vi "Process Messages.vi"(8 "error in (no error)":errorcluster, 11 "Deck in":refnum<class "Deck.lvclass">) -> (0 "error out":errorcluster, 3 "Deck out":refnum<class "Deck.lvclass">)   [LabVIEW 2019, in "Deck.lvclass"]
uses:
  Deck.lvclass
  Deck.lvclass/Deck.ctl
  Libraries/Track Info/Track Info.ctl
  State.ctl
  Packed Libraries/Messaging.lvlibp/Message Cluster.ctl
  Libraries/Track Info/Track Info FGV Enum.ctl
  Packed Libraries/Globals.lvlibp/Constants.vi
  Libraries/Audio File Input/Audio File Input.lvlib
  Packed Libraries/Messaging.lvlibp
  Libraries/User Interface/User Interface.lvlib
  Libraries/Track Info/Track Info.lvlib
  Packed Libraries/Globals.lvlibp
  Packed Libraries/Audio Processing.lvlibp
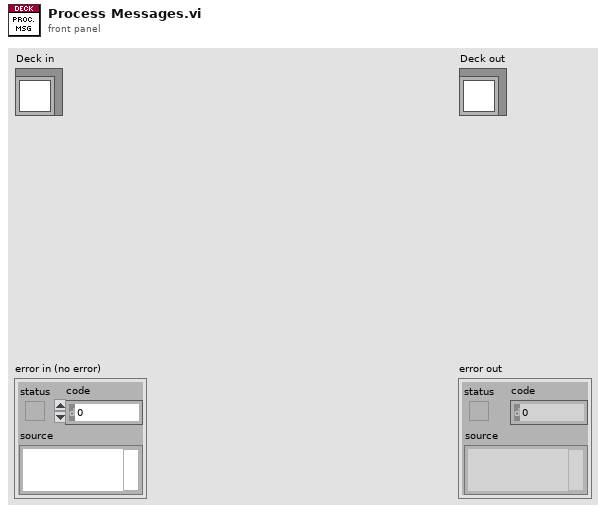
[diagram p1: front panel]
types:
  T1 = typedef "Track Info.lvlib/Track Info.ctl" = cluster{"Path":path, "Length (Samples)":i32, "Channels":i32, "Sample Rate (Hz)":i32, "BPM":dbl, "Cue Points (Samples)":i32[]}
  T2 = typedef "Messaging.lvlibp/Message Cluster.ctl" = cluster{"Event":string, "Source":string, "Target":string, "Data":variant}
  T3 = typedef "Deck.lvclass/State.ctl" = enum16{"No Track", "Loading", "Active", "Scratching", "Brake", "Backspin"}
  T4 = typedef "Track Info.lvlib/Track Info FGV Enum.ctl" = enum16{"Init", "Update Track", "Update Multiple Tracks", "Get Track", "Get Multiple Tracks"}
  T5 = typedef "Audio Processing.lvlibp/Value Properties.ctl" = cluster{"Lower":dbl, "Upper":dbl, "Default":dbl, "Increment":dbl}
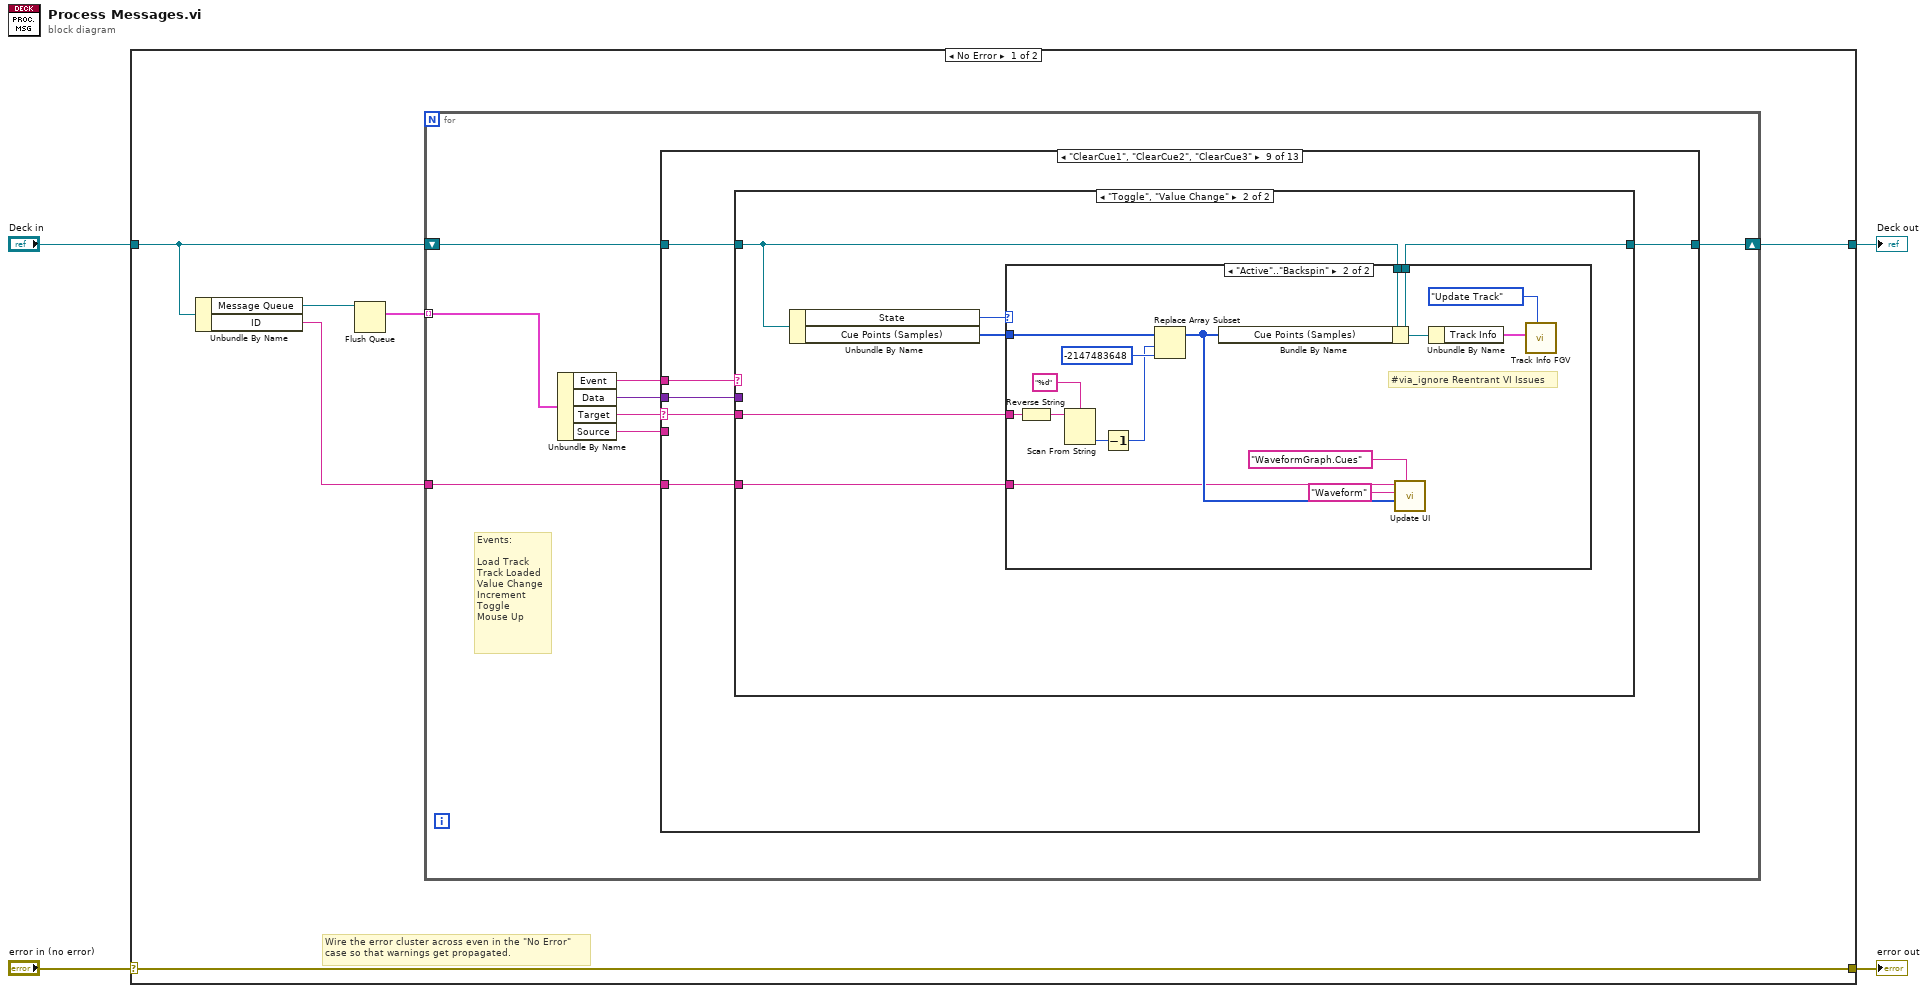
[diagram p0: block diagram]
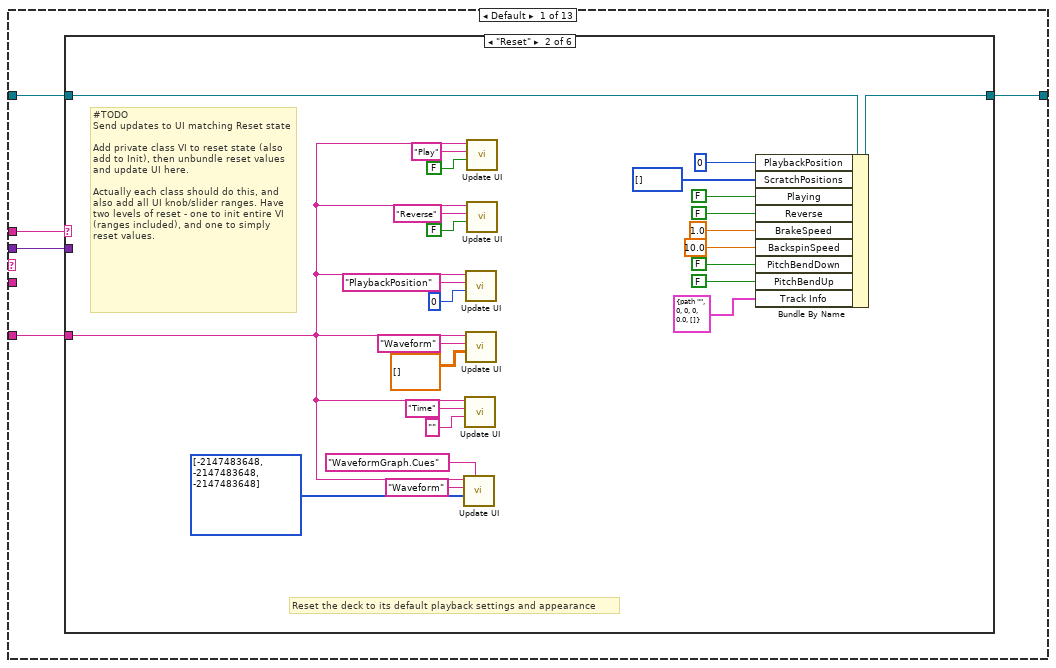
[diagram p2: hidden frame]
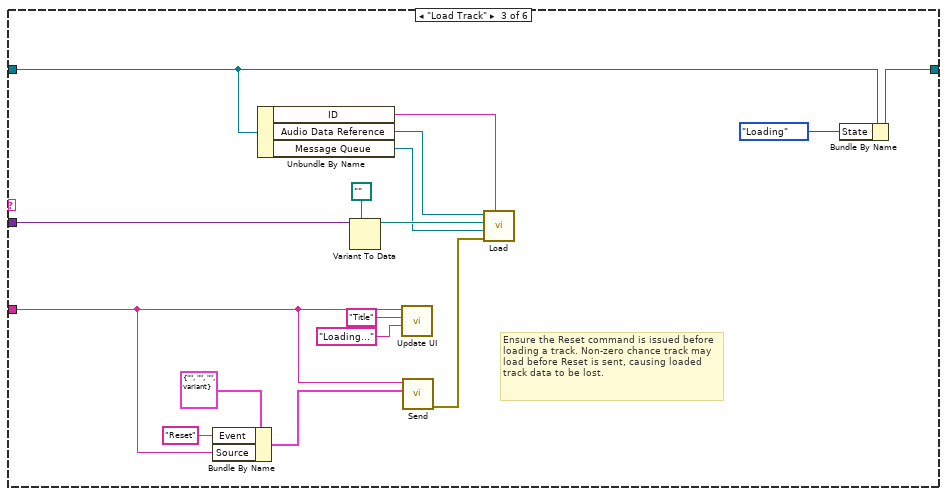
[diagram p4: hidden frame]
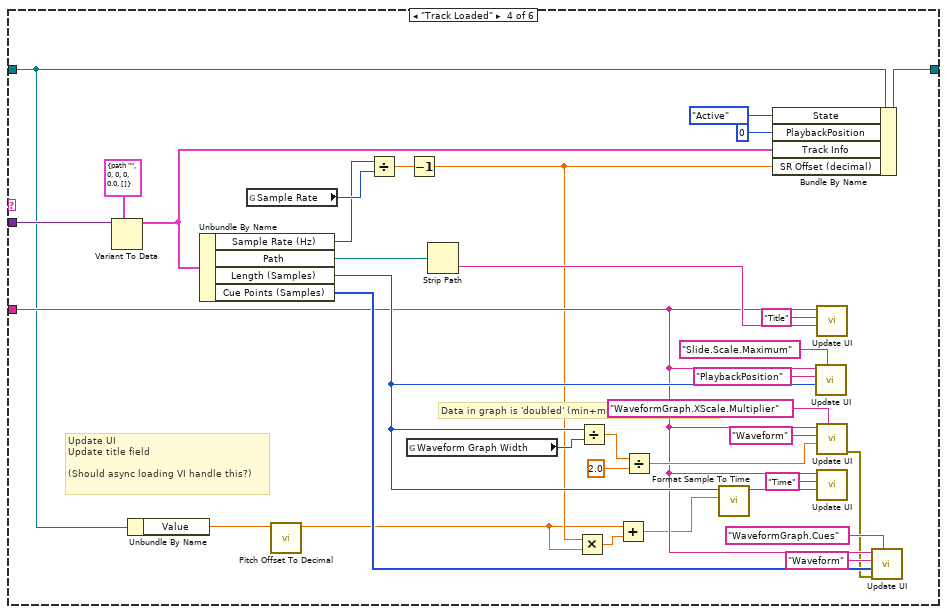
[diagram p5: hidden frame]
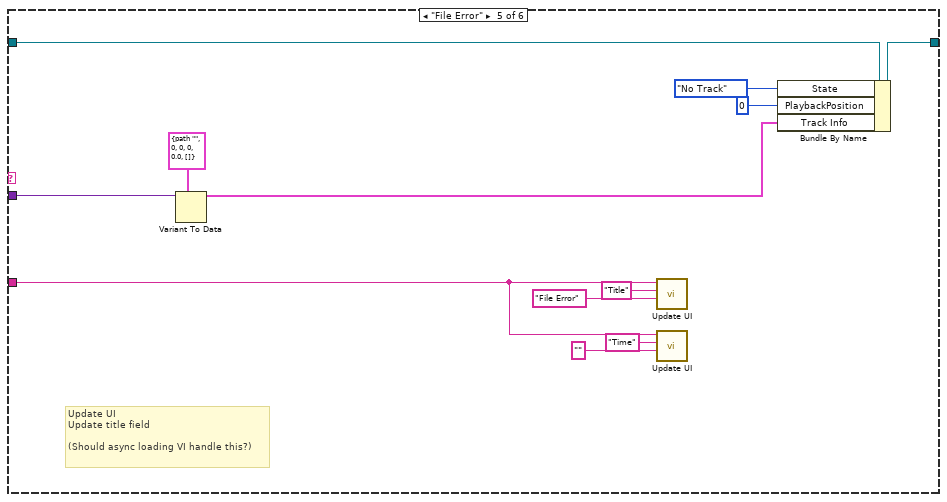
[diagram p6: hidden frame]
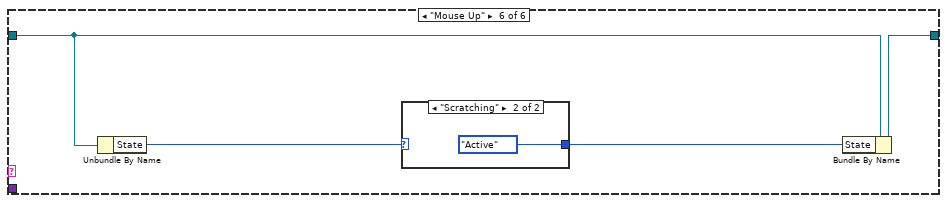
[diagram p7: hidden frame]
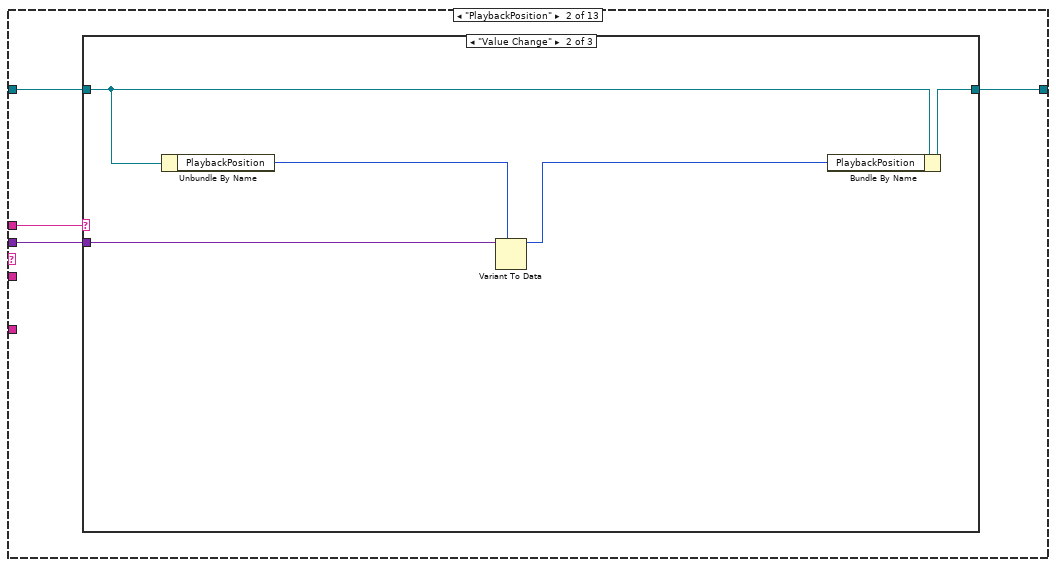
[diagram p9: hidden frame]
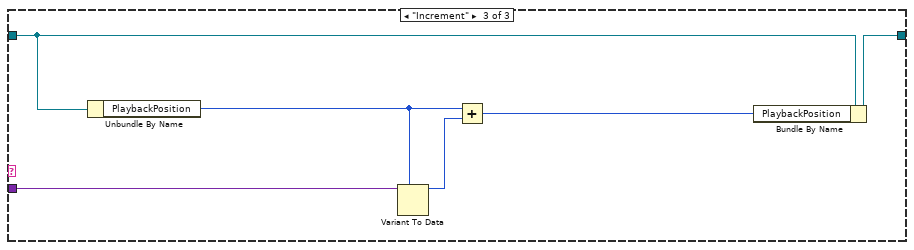
[diagram p11: hidden frame]
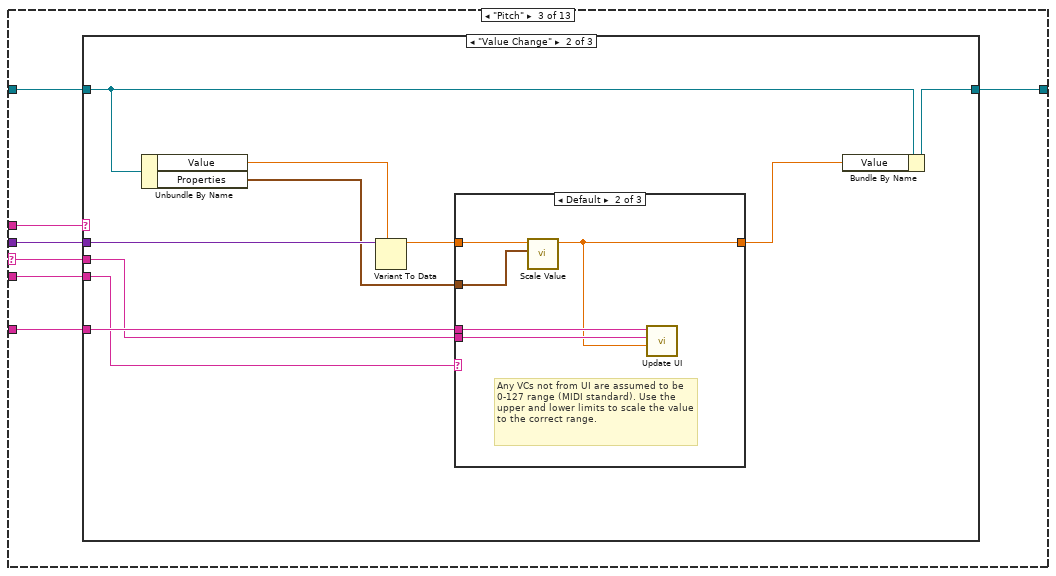
[diagram p12: hidden frame]
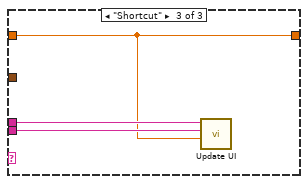
[diagram p15: hidden frame]
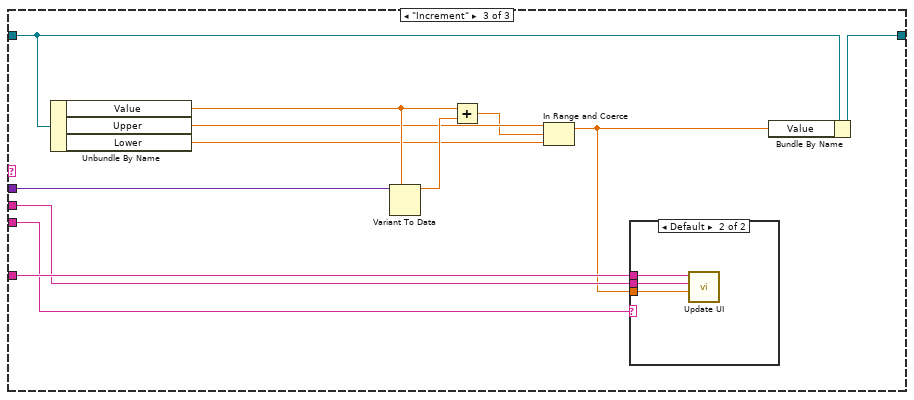
[diagram p16: hidden frame]
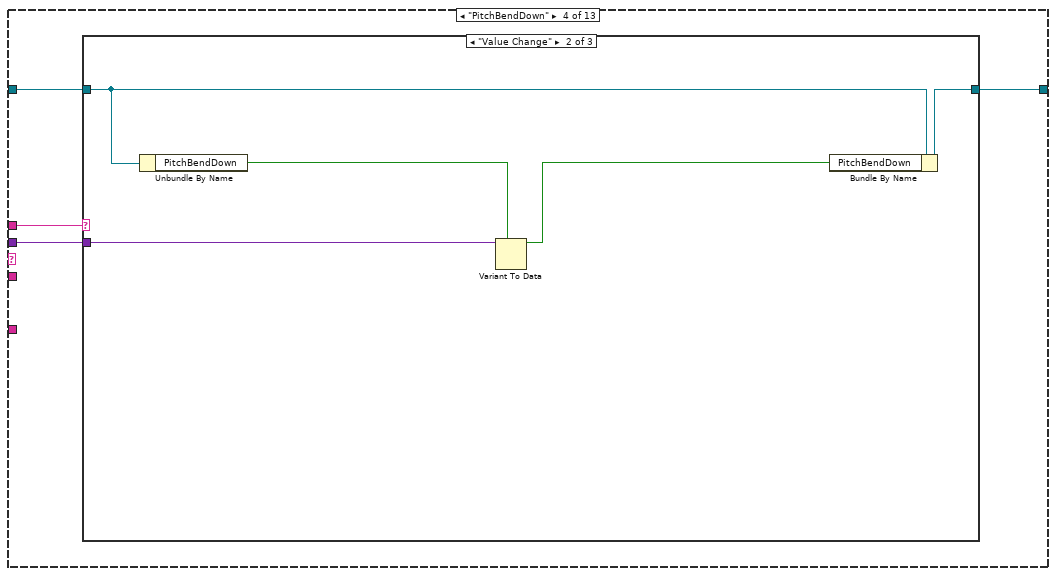
[diagram p18: hidden frame]
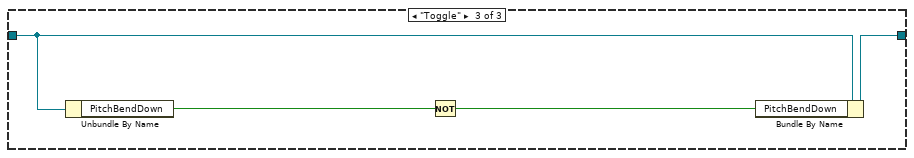
[diagram p20: hidden frame]
diagram:
  n1 = case shown="No Error" "error in (no error)" {
    selector: "error in (no error)" -> [w10 w558]
    tunnel: [w10 w558] -> w3
    tunnel: [w9 w557] -> w1
    tunnel: "Deck in" -> [w8 w557]
    frame No Error {
      # "Wire the error cluster across even in the \"No Error\"\ncase so that warnings get propagated."
      n2 = Unbundle By Name(w8) -> ("Message Queue"=w6:refnum<queue>, "ID"=w7:string)
      n3 = Flush Queue(queue=w6) -> (remaining elements=w5:T2[])  [unwired: 1 in, 2 out]
      n4 = for {
        shift-right: [w16] -> w9
        shift-left: w8 -> [w18]
        tunnel: w7 -> [w14]
        tunnel: w5 -> [w11] mode=indexing
        # "Events:\n\nLoad Track\nTrack Loaded\nValue Change\nIncrement\nToggle\nMouse Up"
        n5 = Unbundle By Name(w11) -> ("Event"=w17:string, "Data"=w15:variant, "Target"=w13:string, "Source"=w12:string)
        n6 = case shown="\"ClearCue1\", \"ClearCue2\", \"ClearCue3\"" w13 {
          selector: w13 -> [_ _ w135 _ _ _ w223 w250 w280 w310 w347 w377 w468]
          tunnel: w18 -> [w23 w121 w140 w179 w193 w207 w227 w254 w284 w314 w352 w381 w472]
          tunnel: w17 -> [w22 w120 w139 w178 w192 w206 w226 w253 w283 w313 w351 w380 w471]
          tunnel: [w21 w119 w138 w177 w191 w205 w225 w252 w282 w312 w350 w379 w470] -> w16
          tunnel: w15 -> [w20 w118 w137 w176 w190 w204 w224 w251 w281 w311 w349 w378 w469]
          tunnel: w14 -> [w19 _ w136 _ _ _ _ w249 w279 w309 w348 w376 w467]
          tunnel: w12 -> [_ _ w134 _ _ _ _ _ _ w308 w346 w375 w466]
          frame Default {
            n7 = case shown="\"Reset\"" w22 {
              tunnel: w23 -> [w24 w42 w58 w71 w109 w112]
              tunnel: [w24 w43 w59 w97 w108 w113] -> w21
              tunnel: w20 -> [_ _ w57 w96 w107 _]
              tunnel: w19 -> [_ w27 w51 w76 w103 _]
              frame Default {
              }
              frame "Reset" {
                # "#TODO\nSend updates to UI matching Reset state\n\nAdd private class VI to reset state (also add to Init), then unbundle reset values and update UI here.\n\nActually each class should do this, and also add all UI knob/slider ranges. Have two levels of reset - one to init entire VI (ranges included), and one to simply reset values."
                # "Reset the deck to its default playback settings and appearance"
                n8 = call "Update UI.vi"("Message (Value Change)"="WaveformGraph.Cues" ("format string"), "Data"=i32[] [-2147483648, -2147483648, -2147483648] ("Cue Points (Samples)"), "Target"="Waveform", "ID"=w27) -> ()  [unwired: 7 in, 1 out]
                n9 = call "Update UI.vi"("Data"="" ("Target"), "Target"="Time", "ID"=w27) -> ()  [unwired: 8 in, 1 out]
                n10 = call "Update UI.vi"("Data"=0, "Target"="PlaybackPosition", "ID"=w27) -> ()  [unwired: 8 in, 1 out]
                n11 = call "Update UI.vi"("Data"=dbl[][] [], "Target"="Waveform", "ID"=w27) -> ()  [unwired: 8 in, 1 out]
                n12 = call "Update UI.vi"("Data"=FALSE ("Playing"), "Target"="Play", "ID"=w27) -> ()  [unwired: 8 in, 1 out]
                n13 = call "Update UI.vi"("Data"=FALSE ("Playing"), "Target"="Reverse", "ID"=w27) -> ()  [unwired: 8 in, 1 out]
                n14 = Bundle By Name(cluster=w42, "PlaybackPosition"=0, "ScratchPositions"=i32[] [], "Playing"=FALSE, "Reverse"=FALSE, "BrakeSpeed"=1.0, "BackspinSpeed"=10.0, "PitchBendDown"=FALSE, "PitchBendUp"=FALSE, "Track Info"=T1 {"Path"=path "", "Length (Samples)"=0, "Channels"=0, "Sample Rate (Hz)"=0, "BPM"=0.0, "Cue Points (Samples)"=[]}) -> (w43:refnum<class "Deck.lvclass">)
              }
              frame "Load Track" {
                # "Ensure the Reset command is issued before loading a track. Non-zero chance track may load before Reset is sent, causing loaded track data to be lost."
                n15 = Bundle By Name(cluster=T2 {"Event"="", "Source"="", "Target"="", "Data"=variant} ("Message"), "Event"="Reset", "Source"=w51) -> (w52:T2)
                n16 = Unbundle By Name(w58) -> ("ID"=w65:string, "Audio Data Reference"=w62:refnum<data-value>, "Message Queue"=w61:refnum<queue>)
                n17 = Variant To Data(type=path "", Variant=w57) -> (data=w64:path)  [unwired: 1 in, 1 out]
                n18 = call "Update UI.vi"("Data"="Loading..." ("Target"), "Target"="Title", "ID"=w51) -> ()  [unwired: 8 in, 1 out]
                n19 = call "Send.vi"("Message"=w52, "Queue Name"=w51) -> ("error out"=w50:errorcluster)  [unwired: 9 in]
                n20 = call "Load.vi"("Deck ID"=w65, "error in (no error)"=w50, "Message Queue"=w61, "Path"=w64, "Audio Data Reference"=w62) -> ()  [unwired: 6 in, 1 out]
                n21 = Bundle By Name(cluster=w58, "State"=State."Loading") -> (w59:refnum<class "Deck.lvclass">)
              }
              frame "Track Loaded" {
                # "Data in graph is 'doubled' (min+max for every point)"
                # "Update UI\nUpdate title field\n\n(Should async loading VI handle this?)"
                n22 = Variant To Data(type=T1 {"Path"=path "", "Length (Samples)"=0, "Channels"=0, "Sample Rate (Hz)"=0, "BPM"=0.0, "Cue Points (Samples)"=[]} ("Track Info"), Variant=w96) -> (data=w94:T1)  [unwired: 1 in, 1 out]
                n23 = Unbundle By Name(w71) -> ("Value"=w70:dbl)
                n24 = Unbundle By Name(w94) -> ("Sample Rate (Hz)"=w72:i32, "Path"=w93:path, "Length (Samples)"=w84:i32, "Cue Points (Samples)"=w77:i32[])
                n25 = global read "Constants.vi" "Sample Rate"() -> (w74:i32)
                n26 = call "Pitch Offset To Decimal.vi"("Pitch Offset (%)"=w70) -> ("Pitch (decimal)"=w67:dbl)  [unwired: 10 in]
                n27 = Divide(x=w72, y=w74) -> (x/y=w73:dbl)
                n28 = global read "Constants.vi" "Waveform Graph Width"() -> (w83:i32)
                n29 = Decrement(x=w73) -> (x-1=w68:dbl)
                n30 = Strip Path(path=w93) -> (name=w92:string)  [unwired: 1 out]
                n31 = Multiply(x=w68, y=w67) -> (x*y=w69:dbl)
                n32 = Divide(x=w84, y=w83) -> (x/y=w82:dbl)
                n33 = Add(x=w67, y=w69) -> (x+y=w66:dbl)
                n34 = Divide(x=w82, y=2.0 ("x")) -> (x/y=w80:dbl)
                n35 = call "Format Sample To Time.vi"("Pitch (decimal) (1)"=w66, "Samples"=w84) -> ("Formatted Time"=w88:string)  [unwired: 9 in]
                n36 = Bundle By Name(cluster=w71, "State"=State."Active", "PlaybackPosition"=0 ("Playback Position (Samples)"), "Track Info"=w94, "SR Offset (decimal)"=w68) -> (w97:refnum<class "Deck.lvclass">)
                n37 = call "Update UI.vi"("Message (Value Change)"="Slide.Scale.Maximum" ("Target"), "Data"=w84, "Target"="PlaybackPosition", "ID"=w76) -> ()  [unwired: 7 in, 1 out]
                n38 = call "Update UI.vi"("Data"=w92, "Target"="Title", "ID"=w76) -> ()  [unwired: 8 in, 1 out]
                n39 = call "Update UI.vi"("Message (Value Change)"="WaveformGraph.XScale.Multiplier" ("Target"), "Data"=w80, "Target"="Waveform", "ID"=w76) -> ("error out"=w75:errorcluster)  [unwired: 7 in]
                n40 = call "Update UI.vi"("Data"=w88, "Target"="Time", "ID"=w76) -> ()  [unwired: 8 in, 1 out]
                n41 = call "Update UI.vi"("Message (Value Change)"="WaveformGraph.Cues" ("format string"), "error in (no error)"=w75, "Data"=w77, "Target"="Waveform", "ID"=w76) -> ()  [unwired: 6 in, 1 out]
              }
              frame "File Error" {
                # "Update UI\nUpdate title field\n\n(Should async loading VI handle this?)"
                n42 = Variant To Data(type=T1 {"Path"=path "", "Length (Samples)"=0, "Channels"=0, "Sample Rate (Hz)"=0, "BPM"=0.0, "Cue Points (Samples)"=[]} ("Track Info"), Variant=w107) -> (data=w105:T1)  [unwired: 1 in, 1 out]
                n43 = call "Update UI.vi"("Data"="File Error" ("Target"), "Target"="Title", "ID"=w103) -> ()  [unwired: 8 in, 1 out]
                n44 = call "Update UI.vi"("Data"="" ("Target"), "Target"="Time", "ID"=w103) -> ()  [unwired: 8 in, 1 out]
                n45 = Bundle By Name(cluster=w109, "State"=State."No Track", "PlaybackPosition"=0 ("Playback Position (Samples)"), "Track Info"=w105) -> (w108:refnum<class "Deck.lvclass">)
              }
              frame "Mouse Up" {
                n46 = Unbundle By Name(w112) -> ("State"=w114:T3)
                n47 = case shown="\"Scratching\"" w114 {
                  selector: w114 -> [w116 _]
                  tunnel: [w116 State."Active" ("State")] -> w115
                  frame Default {
                  }
                  frame "Scratching" {
                  }
                }
                n48 = Bundle By Name(cluster=w112, "State"=w115) -> (w113:refnum<class "Deck.lvclass">)
              }
            }
          }
          frame "PlaybackPosition" {
            n49 = case shown="\"Value Change\"" w120 {
              tunnel: w121 -> [w122 w126 w132]
              tunnel: [w122 w127 w133] -> w119
              tunnel: w118 -> [_ w124 w131]
              frame Default {
              }
              frame "Value Change" {
                n50 = Unbundle By Name(w126) -> ("PlaybackPosition"=w125:i32)
                n51 = Variant To Data(type=w125, Variant=w124) -> (data=w123:i32)  [unwired: 1 in, 1 out]
                n52 = Bundle By Name(cluster=w126, "PlaybackPosition"=w123) -> (w127:refnum<class "Deck.lvclass">)
              }
              frame "Increment" {
                n53 = Unbundle By Name(w132) -> ("PlaybackPosition"=w130:i32)
                n54 = Variant To Data(type=w130, Variant=w131) -> (data=w129:i32)  [unwired: 1 in, 1 out]
                n55 = Add(x=w130, y=w129) -> (x+y=w128:i32)
                n56 = Bundle By Name(cluster=w132, "PlaybackPosition"=w128) -> (w133:refnum<class "Deck.lvclass">)
              }
            }
          }
          frame "Pitch" {
            n57 = case shown="\"Value Change\"" w139 {
              tunnel: w140 -> [w141 w150 w171]
              tunnel: [w141 w151 w172] -> w138
              tunnel: w137 -> [_ w148 w170]
              tunnel: w136 -> [_ w147 w167]
              tunnel: w135 -> [_ w145 w166]
              tunnel: w134 -> [_ w144 w165]
              frame Default {
              }
              frame "Value Change" {
                n58 = Unbundle By Name(w150) -> ("Value"=w149:dbl, "Properties"=w142:T5)
                n59 = Variant To Data(type=w149, Variant=w148) -> (data=w146:dbl)  [unwired: 1 in, 1 out]
                n60 = case shown="Default" w144 {
                  tunnel: w147 -> [_ w157 w160]
                  tunnel: w145 -> [_ w156 w159]
                  tunnel: w146 -> [w152 w153 w158]
                  tunnel: [w152 w154 w158] -> w143
                  tunnel: w142 -> [_ w155 _]
                  frame "UI" {
                    # "VC from UI are assumed to be in range."
                  }
                  frame Default {
                    # "Any VCs not from UI are assumed to be 0-127 range (MIDI standard). Use the upper and lower limits to scale the value to the correct range."
                    n61 = call "Scale Value.vi"("Properties"=w155, "Value"=w153) -> ("Scaled Value"=w154:dbl)  [unwired: 9 in]
                    n62 = call "Update UI.vi"("Data"=w154, "Target"=w156, "ID"=w157) -> ()  [unwired: 8 in, 1 out]
                  }
                  frame "Shortcut" {
                    n63 = call "Update UI.vi"("Data"=w158, "Target"=w159, "ID"=w160) -> ()  [unwired: 8 in, 1 out]
                  }
                }
                n64 = Bundle By Name(cluster=w150, "Value"=w143) -> (w151:refnum<class "Deck.lvclass">)
              }
              frame "Increment" {
                n65 = Unbundle By Name(w171) -> ("Value"=w169:dbl, "Upper"=w164:dbl, "Lower"=w163:dbl)
                n66 = Variant To Data(type=w169, Variant=w170) -> (data=w168:dbl)  [unwired: 1 in, 1 out]
                n67 = Add(x=w169, y=w168) -> (x+y=w162:dbl)
                n68 = In Range and Coerce(upper limit=w164, x=w162, lower limit=w163) -> (coerced(x)=w161:dbl)  [unwired: 1 out]
                n69 = case shown="Default" w165 {
                  tunnel: w167 -> [_ w175]
                  tunnel: w166 -> [_ w174]
                  tunnel: w161 -> [_ w173]
                  frame "UI" {
                  }
                  frame Default {
                    n70 = call "Update UI.vi"("Data"=w173, "Target"=w174, "ID"=w175) -> ()  [unwired: 8 in, 1 out]
                  }
                }
                n71 = Bundle By Name(cluster=w171, "Value"=w161) -> (w172:refnum<class "Deck.lvclass">)
              }
            }
          }
          frame "PitchBendDown" {
            n72 = case shown="\"Value Change\"" w178 {
              tunnel: w179 -> [w180 w184 w188]
              tunnel: [w180 w185 w189] -> w177
              tunnel: w176 -> [_ w182 _]
              frame Default {
              }
              frame "Value Change" {
                n73 = Unbundle By Name(w184) -> ("PitchBendDown"=w183:bool)
                n74 = Variant To Data(type=w183, Variant=w182) -> (data=w181:bool)  [unwired: 1 in, 1 out]
                n75 = Bundle By Name(cluster=w184, "PitchBendDown"=w181) -> (w185:refnum<class "Deck.lvclass">)
              }
              frame "Toggle" {
                n76 = Unbundle By Name(w188) -> ("PitchBendDown"=w187:bool)
                n77 = Not(x=w187) -> (.not. x?=w186:bool)
                n78 = Bundle By Name(cluster=w188, "PitchBendDown"=w186) -> (w189:refnum<class "Deck.lvclass">)
              }
            }
          }
          frame "PitchBendUp" {
            n79 = case shown="\"Value Change\"" w192 {
              tunnel: w193 -> [w194 w198 w202]
              tunnel: [w194 w199 w203] -> w191
              tunnel: w190 -> [_ w196 _]
              frame Default {
              }
              frame "Value Change" {
                n80 = Unbundle By Name(w198) -> ("PitchBendUp"=w197:bool)
                n81 = Variant To Data(type=w197, Variant=w196) -> (data=w195:bool)  [unwired: 1 in, 1 out]
                n82 = Bundle By Name(cluster=w198, "PitchBendUp"=w195) -> (w199:refnum<class "Deck.lvclass">)
              }
              frame "Toggle" {
                n83 = Unbundle By Name(w202) -> ("PitchBendUp"=w201:bool)
                n84 = Not(x=w201) -> (.not. x?=w200:bool)
                n85 = Bundle By Name(cluster=w202, "PitchBendUp"=w200) -> (w203:refnum<class "Deck.lvclass">)
              }
            }
          }
          frame "Jogwheel" {
            n86 = case shown="\"Value Change\"" w206 {
              tunnel: w207 -> [w208 w219]
              tunnel: [w208 w220] -> w205
              tunnel: w204 -> [_ w218]
              frame Default {
              }
              frame "Value Change" {
                n87 = Unbundle By Name(w219) -> ("State"=w217:T3, "ScratchPositions"=w214:i32[], "PlaybackPosition"=w212:i32)
                n88 = Variant To Data(type=w212, Variant=w218) -> (data=w211:i32)  [unwired: 1 in, 1 out]
                n89 = Subtract(x=w214, y=w212) -> (x-y=w215:i32[])
                n90 = case shown="\"Active\"" w217 {
                  selector: w217 -> [w221 _]
                  tunnel: [w221 State."Scratching" ("State")] -> w216
                  frame Default {
                  }
                  frame "Active" {
                  }
                }
                n91 = Add Array Elements(numeric array=w215) -> (sum=w213:i32)
                n92 = Compound Arithmetic op=ADD(w213, w212, w211) -> (w210:i32)
                n93 = Build Array(w210) -> (w209:i32[])
                n94 = Bundle By Name(cluster=w219, "State"=w216, "ScratchPositions"=w209) -> (w220:refnum<class "Deck.lvclass">)
              }
            }
          }
          frame "Cue1", "Cue2", "Cue3" {
            n95 = case shown="\"Toggle\", \"Value Change\"" w226 {
              tunnel: w227 -> [w228 w232]
              tunnel: [w228 w233] -> w225
              tunnel: w224 -> [_ _]
              tunnel: w223 -> [_ w230]
              frame Default {
              }
              frame "Toggle", "Value Change" {
                n96 = Unbundle By Name(w232) -> ("State"=w229:T3, "Cue Points (Samples)"=w231:i32[])
                n97 = case shown="\"Active\"..\"Backspin\"" w229 {
                  tunnel: [w234 w244] -> w233
                  tunnel: w232 -> [w234 w243]
                  tunnel: w231 -> [_ w242]
                  tunnel: w230 -> [_ w237]
                  frame Default {
                  }
                  frame "Active".."Backspin" {
                    n98 = Reverse String(1:w237) -> (0:w239:string)
                    n99 = Scan From String(format string="%d", input string=w239) -> (output 1=w236:i32)  [unwired: 3 in, 3 out]
                    n100 = Decrement(x=w236) -> (x-1=w235:i32)
                    n101 = Index Array(array=w242, index=w235) -> (element=w240:i32)
                    n102 = Greater Or Equal To 0?(x=w240) -> (x >= 0?=w241:bool)
                    n103 = case shown="True" w241 {
                      tunnel: [w245 w248] -> w244
                      tunnel: w243 -> [w245 w247]
                      tunnel: w240 -> [_ w246]
                      frame False {
                      }
                      frame True {
                        n104 = Bundle By Name(cluster=w247, "PlaybackPosition"=w246) -> (w248:refnum<class "Deck.lvclass">)
                      }
                    }
                  }
                }
              }
            }
          }
          frame "SetCue1", "SetCue2", "SetCue3" {
            n105 = case shown="\"Toggle\", \"Value Change\"" w253 {
              tunnel: w254 -> [w255 w262]
              tunnel: [w255 w260] -> w252
              tunnel: w251 -> [_ _]
              tunnel: w250 -> [_ w258]
              tunnel: w249 -> [_ w257]
              frame Default {
              }
              frame "Toggle", "Value Change" {
                n106 = Unbundle By Name(w262) -> ("State"=w256:T3, "PlaybackPosition"=w261:i32, "Cue Points (Samples)"=w259:i32[])
                n107 = case shown="\"Active\"..\"Backspin\"" w256 {
                  tunnel: w262 -> [w263 w278]
                  tunnel: w261 -> [_ w277]
                  tunnel: [w263 w274] -> w260
                  tunnel: w259 -> [_ w273]
                  tunnel: w258 -> [_ w272]
                  tunnel: w257 -> [_ w265]
                  frame Default {
                  }
                  frame "Active".."Backspin" {
                    # "#via_ignore Reentrant VI Issues"
                    n108 = Reverse String(1:w272) -> (0:w271:string)
                    n109 = Scan From String(format string="%d", input string=w271) -> (output 1=w269:i32)  [unwired: 3 in, 3 out]
                    n110 = Decrement(x=w269) -> (x-1=w268:i32)
                    n111 = Replace Array Subset(array=w273, new element=w277, index=w268) -> (w266:i32[])
                    n112 = Bundle By Name(cluster=w278, "Cue Points (Samples)"=w266) -> (w274:refnum<class "Deck.lvclass">)
                    n113 = call "Update UI.vi"("Message (Value Change)"="WaveformGraph.Cues" ("format string"), "Data"=w266, "Target"="Waveform", "ID"=w265) -> ()  [unwired: 7 in, 1 out]
                    n114 = Unbundle By Name(w274) -> ("Track Info"=w276:T1)
                    n115 = call "Track Info FGV.vi"("Track Info FGV Enum"=Track_Info_FGV_Enum."Update Track", "Track Info In"=w276) -> ()  [unwired: 6 in, 4 out]
                  }
                }
              }
            }
          }
          frame "ClearCue1", "ClearCue2", "ClearCue3" {
            n116 = case shown="\"Toggle\", \"Value Change\"" w283 {
              tunnel: w284 -> [w285 w291]
              tunnel: [w285 w288] -> w282
              tunnel: w281 -> [_ _]
              tunnel: w280 -> [_ w289]
              tunnel: w279 -> [_ w287]
              frame Default {
              }
              frame "Toggle", "Value Change" {
                n117 = Unbundle By Name(w291) -> ("State"=w286:T3, "Cue Points (Samples)"=w290:i32[])
                n118 = case shown="\"Active\"..\"Backspin\"" w286 {
                  tunnel: w291 -> [w292 w307]
                  tunnel: w290 -> [_ w306]
                  tunnel: w289 -> [_ w300]
                  tunnel: [w292 w297] -> w288
                  tunnel: w287 -> [_ w293]
                  frame Default {
                  }
                  frame "Active".."Backspin" {
                    # "#via_ignore Reentrant VI Issues"
                    n119 = Reverse String(1:w300) -> (0:w302:string)
                    n120 = Scan From String(format string="%d", input string=w302) -> (output 1=w299:i32)  [unwired: 3 in, 3 out]
                    n121 = Decrement(x=w299) -> (x-1=w298:i32)
                    n122 = Replace Array Subset(array=w306, new element=-2147483648 ("new element/subarray"), index=w298) -> (w294:i32[])
                    n123 = Bundle By Name(cluster=w307, "Cue Points (Samples)"=w294) -> (w297:refnum<class "Deck.lvclass">)
                    n124 = call "Update UI.vi"("Message (Value Change)"="WaveformGraph.Cues" ("format string"), "Data"=w294, "Target"="Waveform", "ID"=w293) -> ()  [unwired: 7 in, 1 out]
                    n125 = Unbundle By Name(w297) -> ("Track Info"=w304:T1)
                    n126 = call "Track Info FGV.vi"("Track Info FGV Enum"=Track_Info_FGV_Enum."Update Track", "Track Info In"=w304) -> ()  [unwired: 6 in, 4 out]
                  }
                }
              }
            }
          }
          frame "Play" {
            n127 = case shown="\"Value Change\"" w313 {
              tunnel: w314 -> [w315 w323 w338]
              tunnel: [w315 w324 w339] -> w312
              tunnel: w311 -> [_ w321 _]
              tunnel: w310 -> [_ w319 w335]
              tunnel: w309 -> [_ w318 w334]
              tunnel: w308 -> [_ w317 w332]
              frame Default {
              }
              frame "Value Change" {
                n128 = Unbundle By Name(w323) -> ("State"=w322:T3, "Playing"=w320:bool)
                n129 = case shown="\"Active\"..\"Backspin\"" w322 {
                  tunnel: w321 -> [_ w331]
                  tunnel: w320 -> [w328 w330]
                  tunnel: [w328 w329] -> w316
                  frame Default {
                  }
                  frame "Active".."Backspin" {
                    n130 = Variant To Data(type=w330, Variant=w331) -> (data=w329:bool)  [unwired: 1 in, 1 out]
                  }
                }
                n131 = case shown="Default" w317 {
                  tunnel: w318 -> [_ w327]
                  tunnel: w319 -> [_ w326]
                  tunnel: w316 -> [_ w325]
                  frame "UI" {
                  }
                  frame Default {
                    n132 = call "Update UI.vi"("Data"=w325, "Target"=w326, "ID"=w327) -> ()  [unwired: 8 in, 1 out]
                  }
                }
                n133 = Bundle By Name(cluster=w323, "Playing"=w316) -> (w324:refnum<class "Deck.lvclass">)
              }
              frame "Toggle" {
                n134 = Unbundle By Name(w338) -> ("State"=w337:T3, "Playing"=w336:bool)
                n135 = case shown="\"Active\"..\"Backspin\"" w337 {
                  tunnel: w336 -> [w343 w345]
                  tunnel: [w343 w344] -> w333
                  frame Default {
                  }
                  frame "Active".."Backspin" {
                    n136 = Not(x=w345) -> (.not. x?=w344:bool)
                  }
                }
                n137 = case shown="Default" w332 {
                  tunnel: w334 -> [_ w342]
                  tunnel: w335 -> [_ w341]
                  tunnel: w333 -> [_ w340]
                  frame "UI" {
                  }
                  frame Default {
                    n138 = call "Update UI.vi"("Data"=w340, "Target"=w341, "ID"=w342) -> ()  [unwired: 8 in, 1 out]
                  }
                }
                n139 = Bundle By Name(cluster=w338, "Playing"=w333) -> (w339:refnum<class "Deck.lvclass">)
              }
            }
          }
          frame "Reverse" {
            n140 = case shown="\"Value Change\"" w351 {
              tunnel: w352 -> [w353 w360 w370]
              tunnel: [w353 w361 w371] -> w350
              tunnel: w349 -> [_ w359 _]
              tunnel: w348 -> [_ w357 w367]
              tunnel: w347 -> [_ w356 w366]
              tunnel: w346 -> [_ w355 w365]
              frame Default {
              }
              frame "Value Change" {
                n141 = Unbundle By Name(w360) -> ("Reverse"=w358:bool)
                n142 = Variant To Data(type=w358, Variant=w359) -> (data=w354:bool)  [unwired: 1 in, 1 out]
                n143 = case shown="Default" w355 {
                  tunnel: w357 -> [_ w364]
                  tunnel: w356 -> [_ w363]
                  tunnel: w354 -> [_ w362]
                  frame "UI" {
                  }
                  frame Default {
                    n144 = call "Update UI.vi"("Data"=w362, "Target"=w363, "ID"=w364) -> ()  [unwired: 8 in, 1 out]
                  }
                }
                n145 = Bundle By Name(cluster=w360, "Reverse"=w354) -> (w361:refnum<class "Deck.lvclass">)
              }
              frame "Toggle" {
                n146 = Unbundle By Name(w370) -> ("Reverse"=w369:bool)
                n147 = Not(x=w369) -> (.not. x?=w368:bool)
                n148 = case shown="Default" w365 {
                  tunnel: w367 -> [_ w374]
                  tunnel: w366 -> [_ w373]
                  tunnel: w368 -> [_ w372]
                  frame "UI" {
                  }
                  frame Default {
                    n149 = call "Update UI.vi"("Data"=w372, "Target"=w373, "ID"=w374) -> ()  [unwired: 8 in, 1 out]
                  }
                }
                n150 = Bundle By Name(cluster=w370, "Reverse"=w368) -> (w371:refnum<class "Deck.lvclass">)
              }
            }
          }
          frame "Brake" {
            n151 = case shown="\"Toggle\"" w380 {
              tunnel: w381 -> [w382 w395 w444]
              tunnel: [w382 w396 w445] -> w379
              tunnel: w378 -> [_ w391 _]
              tunnel: w377 -> [_ w387 w439]
              tunnel: w376 -> [_ w386 w438]
              tunnel: w375 -> [_ _ _]
              frame Default {
              }
              frame "Value Change" {
                n152 = Unbundle By Name(w395) -> ("Playing"=w388:bool, "State"=w389:T3, "BrakeSpeed"=w394:dbl)
                n153 = Variant To Data(type=FALSE, Variant=w391) -> (data=w390:bool)  [unwired: 1 in, 1 out]
                n154 = case shown="\"Brake\"" w389 {
                  selector: w389 -> [w397 w399 w417]
                  tunnel: w390 -> [_ w401 w419]
                  tunnel: w394 -> [w398 w402 w420]
                  tunnel: [w398 w403 w421] -> w393
                  tunnel: [w397 w404 w422] -> w385
                  tunnel: w388 -> [_ w400 w418]
                  frame Default {
                  }
                  frame "Active" {
                    n155 = case shown="True" w400 {
                      selector: w400 -> [_ w409]
                      tunnel: [w405 w412] -> w404
                      tunnel: [w406 w411] -> w403
                      tunnel: w402 -> [w406 w410]
                      tunnel: w401 -> [_ w408]
                      tunnel: w399 -> [w405 w407]
                      frame False {
                      }
                      frame True {
                        n156 = case shown="True" w408 {
                          tunnel: [w413 State."Brake" ("State")] -> w412
                          tunnel: [w414 1.0 ("BrakeSpeed")] -> w411
                          tunnel: w410 -> [w414 _]
                          tunnel: w409 -> [_ _]
                          tunnel: w407 -> [w413 _]
                          frame False {
                          }
                          frame True {
                          }
                        }
                      }
                    }
                  }
                  frame "Brake" {
                    n157 = case shown="True" w418 {
                      selector: w418 -> [_ w427]
                      tunnel: [w423 w430] -> w422
                      tunnel: [w424 w429] -> w421
                      tunnel: w420 -> [w424 w428]
                      tunnel: w419 -> [_ w426]
                      tunnel: w417 -> [w423 w425]
                      frame False {
                      }
                      frame True {
                        n158 = case shown="False" w426 {
                          tunnel: [State."Active" ("State") w433] -> w430
                          tunnel: [1.0 ("BrakeSpeed") w434] -> w429
                          tunnel: w428 -> [_ w434]
                          tunnel: w427 -> [_ _]
                          tunnel: w425 -> [_ w433]
                          frame False {
                          }
                          frame True {
                          }
                        }
                      }
                    }
                  }
                }
                n159 = Equal?(x=w385, y=State."Brake") -> (x = y?=w383:bool)
                n160 = Bundle By Name(cluster=w395, "State"=w385, "BrakeSpeed"=w393) -> (w396:refnum<class "Deck.lvclass">)
                n161 = call "Update UI.vi"("Data"=w383, "Target"=w387, "ID"=w386) -> ()  [unwired: 8 in, 1 out]
              }
              frame "Toggle" {
                n162 = Unbundle By Name(w444) -> ("Playing"=w440:bool, "State"=w441:T3, "BrakeSpeed"=w443:dbl)
                n163 = case shown="\"Active\"" w441 {
                  selector: w441 -> [w446 w448 w457]
                  tunnel: w443 -> [w447 w450 w459]
                  tunnel: [w447 w451 w460] -> w442
                  tunnel: [w446 w452 w461] -> w437
                  tunnel: w440 -> [_ w449 w458]
                  frame Default {
                  }
                  frame "Active" {
                    n164 = case shown="True" w449 {
                      tunnel: [w453 State."Brake" ("State")] -> w452
                      tunnel: [w454 1.0 ("BrakeSpeed")] -> w451
                      tunnel: w450 -> [w454 _]
                      tunnel: w448 -> [w453 _]
                      frame False {
                      }
                      frame True {
                      }
                    }
                  }
                  frame "Brake" {
                    n165 = case shown="True" w458 {
                      tunnel: [w462 State."Active" ("State")] -> w461
                      tunnel: [w463 1.0 ("BrakeSpeed")] -> w460
                      tunnel: w459 -> [w463 _]
                      tunnel: w457 -> [w462 _]
                      frame False {
                      }
                      frame True {
                      }
                    }
                  }
                }
                n166 = Equal?(x=w437, y=State."Brake" ("State")) -> (x = y?=w435:bool)
                n167 = Bundle By Name(cluster=w444, "State"=w437, "BrakeSpeed"=w442) -> (w445:refnum<class "Deck.lvclass">)
                n168 = call "Update UI.vi"("Data"=w435, "Target"=w439, "ID"=w438) -> ()  [unwired: 8 in, 1 out]
              }
            }
          }
          frame "Backspin" {
            n169 = case shown="\"Toggle\"" w471 {
              tunnel: w472 -> [w473 w486 w535]
              tunnel: [w473 w487 w536] -> w470
              tunnel: w469 -> [_ w482 _]
              tunnel: w468 -> [_ w478 w530]
              tunnel: w467 -> [_ w477 w529]
              tunnel: w466 -> [_ _ _]
              frame Default {
              }
              frame "Value Change" {
                n170 = Unbundle By Name(w486) -> ("Playing"=w479:bool, "State"=w480:T3, "BackspinSpeed"=w485:dbl)
                n171 = Variant To Data(type=FALSE, Variant=w482) -> (data=w481:bool)  [unwired: 1 in, 1 out]
                n172 = case shown="\"Backspin\"" w480 {
                  selector: w480 -> [w488 w490 w508]
                  tunnel: w481 -> [_ w492 w510]
                  tunnel: w485 -> [w489 w493 w511]
                  tunnel: [w489 w494 w512] -> w484
                  tunnel: [w488 w495 w513] -> w476
                  tunnel: w479 -> [_ w491 w509]
                  frame Default {
                  }
                  frame "Active" {
                    n173 = case shown="True" w491 {
                      selector: w491 -> [_ w500]
                      tunnel: [w496 w503] -> w495
                      tunnel: [w497 w502] -> w494
                      tunnel: w493 -> [w497 w501]
                      tunnel: w492 -> [_ w499]
                      tunnel: w490 -> [w496 w498]
                      frame False {
                      }
                      frame True {
                        n174 = case shown="True" w499 {
                          tunnel: [w504 State."Backspin" ("State")] -> w503
                          tunnel: [w505 5.0 ("BrakeSpeed")] -> w502
                          tunnel: w501 -> [w505 _]
                          tunnel: w500 -> [_ _]
                          tunnel: w498 -> [w504 _]
                          frame False {
                          }
                          frame True {
                          }
                        }
                      }
                    }
                  }
                  frame "Backspin" {
                    n175 = case shown="True" w509 {
                      selector: w509 -> [_ w518]
                      tunnel: [w514 w521] -> w513
                      tunnel: [w515 w520] -> w512
                      tunnel: w511 -> [w515 w519]
                      tunnel: w510 -> [_ w517]
                      tunnel: w508 -> [w514 w516]
                      frame False {
                      }
                      frame True {
                        n176 = case shown="False" w517 {
                          tunnel: [State."Active" ("State") w524] -> w521
                          tunnel: [5.0 ("BrakeSpeed") w525] -> w520
                          tunnel: w519 -> [_ w525]
                          tunnel: w518 -> [_ _]
                          tunnel: w516 -> [_ w524]
                          frame False {
                          }
                          frame True {
                          }
                        }
                      }
                    }
                  }
                }
                n177 = Equal?(x=w476, y=State."Backspin") -> (x = y?=w474:bool)
                n178 = Bundle By Name(cluster=w486, "State"=w476, "BackspinSpeed"=w484) -> (w487:refnum<class "Deck.lvclass">)
                n179 = call "Update UI.vi"("Data"=w474, "Target"=w478, "ID"=w477) -> ()  [unwired: 8 in, 1 out]
              }
              frame "Toggle" {
                n180 = Unbundle By Name(w535) -> ("Playing"=w531:bool, "State"=w532:T3, "BackspinSpeed"=w534:dbl)
                n181 = case shown="\"Active\"" w532 {
                  selector: w532 -> [w537 w539 w548]
                  tunnel: w534 -> [w538 w541 w550]
                  tunnel: [w538 w542 w551] -> w533
                  tunnel: [w537 w543 w552] -> w528
                  tunnel: w531 -> [_ w540 w549]
                  frame Default {
                  }
                  frame "Active" {
                    n182 = case shown="True" w540 {
                      tunnel: [w544 State."Backspin" ("State")] -> w543
                      tunnel: [w545 5.0 ("BrakeSpeed")] -> w542
                      tunnel: w541 -> [w545 _]
                      tunnel: w539 -> [w544 _]
                      frame False {
                      }
                      frame True {
                      }
                    }
                  }
                  frame "Backspin" {
                    n183 = case shown="True" w549 {
                      tunnel: [w553 State."Active" ("State")] -> w552
                      tunnel: [w554 5.0 ("BrakeSpeed")] -> w551
                      tunnel: w550 -> [w554 _]
                      tunnel: w548 -> [w553 _]
                      frame False {
                      }
                      frame True {
                      }
                    }
                  }
                }
                n184 = Equal?(x=w528, y=State."Backspin" ("State")) -> (x = y?=w526:bool)
                n185 = Bundle By Name(cluster=w535, "State"=w528, "BackspinSpeed"=w533) -> (w536:refnum<class "Deck.lvclass">)
                n186 = call "Update UI.vi"("Data"=w526, "Target"=w530, "ID"=w529) -> ()  [unwired: 8 in, 1 out]
              }
            }
          }
        }
      }
    }
    frame Error {
    }
  }
  "error out" <- w3
  "Deck out" <- w1
